vi "LabVIEW.Main.API_Test.vi"(7 "Chose Server":string, 8 "error in (no error)":errorcluster caption="Fehler (Eingang, kein Fehler)", 11 "result_folder_path":string) -> (0 "error out":errorcluster, 2 "Message_local_save":string, 3 "Message_report":string)   [LabVIEW 2026]
uses:
  LabVIEW.Type Definitions/LabVIEW.HTTPs_Client.Command.ctl
  LabVIEW.Type Definitions/LabVIEW.HTTPs_Client.Test_Group.Command.ctl
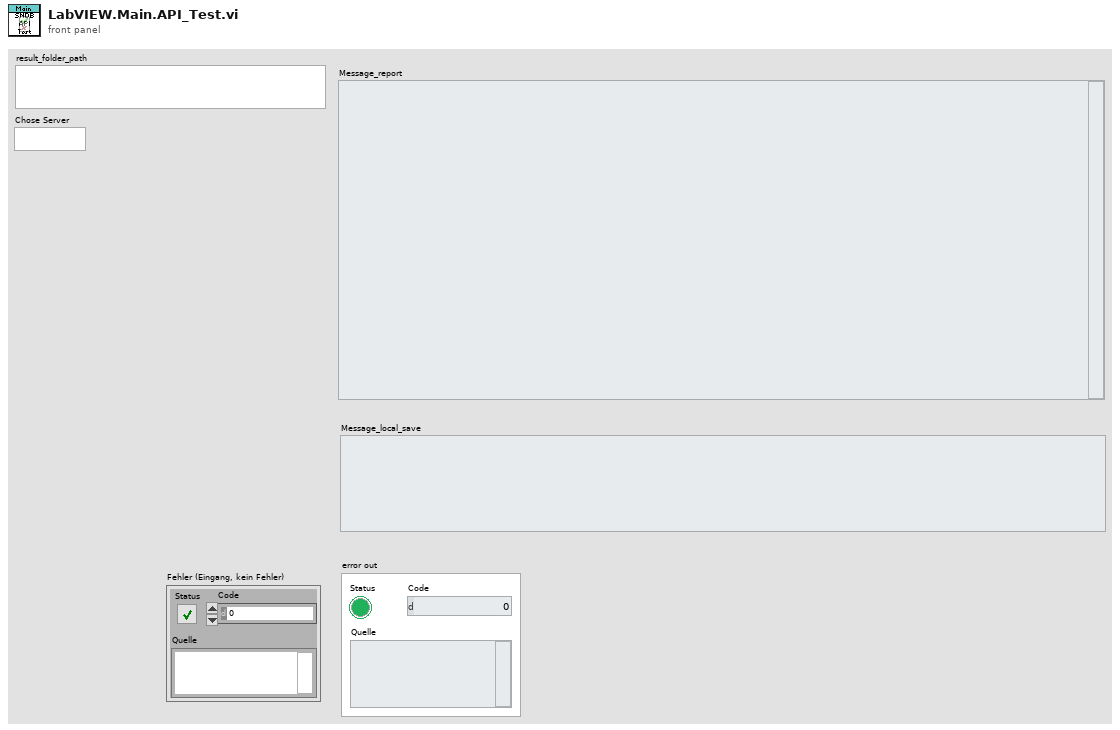
[diagram p1: front panel]
types:
  T1 = typedef "LabVIEW.HTTPs_Client.Command.ctl" = enum16{"Initialize HTTPS", "Authentication: Creat a token", "Authentication: Get all tokens", "Authentication: Revoke the token", "Label: Creat a label configuration", "Label: Get all configured labels", "Label: Update the label configuration", "Label: Delete the label configuration", "Label: Creat a colour ribbon", "Label: Update the colour ribbon", "Label: Get all colour ribbons", "Label: Delete the colour ribbon", "Label: Creat a label tape", "Label: Update the label tape", "Label: Get all label tapes", "Label: Delete the label tape", "Label: Get all label parameters", "Product: Get all product informations", "Product: Get all reading steps", "Seriennummer: Update the info text", "Seriennummer: Set all step states open", "Seriennummer: Update step states", "Seriennummer: Get data and steps", "Seriennummer: Get all label configurations", "Seriennummer: Create a text report(Prüfbericht)", "Seriennummer: Get the text report(Prüfbericht)", "Seriennummer: Delete the text report(Prüfbericht)", "Seriennummer: Upload a document(txt file)", "Seriennummer: Get the document", "Seriennummer: Get the document thumbnail", "Seriennummer: Delete the document", "Seriennummer: Bulk lookup", "Vorgang: Update the description text", "Vorgang: Migrate serial numbers to a Vorgang", "Vorgang: Migrate serial numbers to a product revision", "Vorgang: Update step states", "Vorgang: Create test reports(Prüfprotokoll)", "Vorgang: Get basic data", "Vorgang: Get serial number data and steps", "Vorgang: Get all serial numbers", "Vorgang: Generate a CSV file", "Vorgang: Generate an XLSX file", "Vorgang: Get a CSV file(Fertigmeldung report)", "Fertigmeldung: Create a Fertigmeldung", "Fertigmeldung: Revert the Fertigmeldung", "User: Get all users", "User: Update an user", "User: Get a single user", "User: Get all user roles", "User: Update a user role", "User: Get a single user role", "User: Get all permissions", "Search: Get Vorgang/Produkt combinations", "Search: Get Vorgang/Produkt/SN combinations", "Search: Get Seriennummern by Vorgang and Produkt", "Search: Lookup Vorgang", "MAC addresses: Get all reserved MAC addresses", "MAC addresses: Get the most recently reserved MAC addresses", "MAC addresses: Get data for a MAC address", "MAC addresses: Reserve MAC addresses for a Seriennummer", "MAC addresses: Mark a reserved MAC address as flashed", "Product: Get possible steps", "Product: Get all products", "Product: Create a new product", "Product: Update a product's data", "Product: Get next product IDs", "Product: Delete a product", "Product properties: Get all product property types", "Search: Find production plan", "Search: Find production plan arrangement", "Health check: Health check", "Deinitialize HTTPs"}
  T2 = typedef "LabVIEW.HTTPs_Client.Test_Group.Command.ctl" = enum16{"No Command", " Test Authentication in the beginning", "Test Label", "Test Seriennummer", "Test Vorgang/Fertigung/Search", "Test User/Role/Permission", "Test MAC addresses", "Test Product/Product properties", "Test Health check", " Test Authentication at the end"}
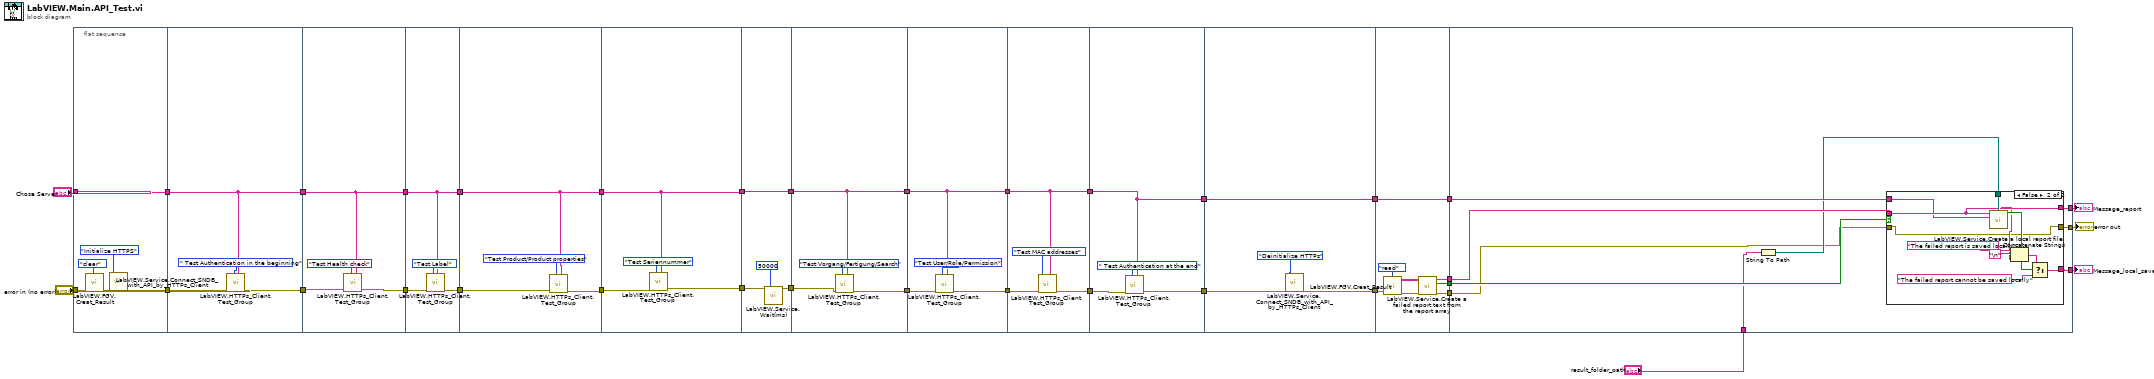
[diagram p0: block diagram]
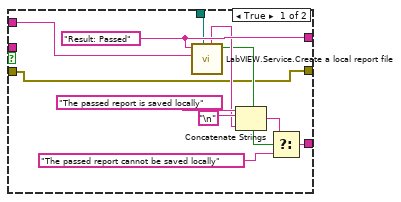
[diagram p2: hidden frame]
diagram:
  n1 = flat-sequence {
    tunnel: "error in (no error)" -> [w36]
    tunnel: [w39] -> w33
    tunnel: [w35] -> w19
    tunnel: "Chose Server" -> [w35]
    tunnel: w33 -> [w43]
    tunnel: [w42] -> w8
    tunnel: w19 -> [w41]
    tunnel: [w41] -> w6
    tunnel: w8 -> [w48]
    tunnel: [w47] -> w7
    tunnel: w6 -> [w45]
    tunnel: [w45] -> w5
    tunnel: w7 -> [w51]
    tunnel: [w50] -> w4
    tunnel: w5 -> [w49]
    tunnel: [w49] -> w2
    tunnel: w4 -> [w56]
    tunnel: [w55] -> w3
    tunnel: w2 -> [w53]
    tunnel: [w53] -> w1
    tunnel: w3 -> [w60]
    tunnel: [w59] -> w32
    tunnel: w1 -> [w58]
    tunnel: [w58] -> w17
    tunnel: w32 -> [w64]
    tunnel: [w63] -> w31
    tunnel: w17 -> [w61]
    tunnel: [w61] -> w16
    tunnel: w31 -> [w68]
    tunnel: [w67] -> w30
    tunnel: w16 -> [w65]
    tunnel: [w65] -> w15
    tunnel: w30 -> [w71]
    tunnel: [w70] -> w29
    tunnel: w15 -> [w69]
    tunnel: [w69] -> w14
    tunnel: w29 -> [w75]
    tunnel: [w74] -> w28
    tunnel: w14 -> [w73]
    tunnel: [w73] -> w13
    tunnel: w28 -> [w79]
    tunnel: [w78] -> w27
    tunnel: w13 -> [w77]
    tunnel: [w77] -> w10
    tunnel: w27 -> [w84]
    tunnel: [w82] -> w26
    tunnel: [w81] -> w11
    tunnel: w10 -> [w81]
    tunnel: w26 -> [w89]
    tunnel: [w88] -> w25
    tunnel: [w87] -> w24
    tunnel: [w86] -> w23
    tunnel: [w85] -> w12
    tunnel: w11 -> [w85]
    tunnel: w25 -> [w93]
    tunnel: w24 -> [w97]
    tunnel: w23 -> [w98]
    tunnel: [w101] -> w22
    tunnel: [w100] -> w21
    tunnel: [w99] -> w20
    tunnel: w12 -> [w96]
    tunnel: "result_folder_path" -> [w94]
    frame #0 {
      n2 = call "LabVIEW.FGV.Creat_Result.vi"("Command"=enum16{"write", "read", "clear"}."clear", "error in (no error)"=w36) -> ("error out"=w37:errorcluster)  [unwired: 8 in, 1 out]
      n3 = call "LabVIEW.Service.Connect_SNDB_with_API_by_HTTPs_Client.vi"("error in (no error)"=w37, "Command"=LabVIEW.HTTPs_Client.Command."Initialize HTTPS") -> ("error out"=w39:errorcluster)  [unwired: 15 in, 10 out]
    }
    frame #1 {
      n4 = call "LabVIEW.HTTPs_Client.Test_Group.vi"("Chose Server"=w41, "Command"=LabVIEW.HTTPs_Client.Test_Group.Command." Test Authentication in the beginning", "Fehler (Eingang, kein Fehler)"=w43) -> ("Fehler (Ausgang)"=w42:errorcluster)  [unwired: 8 in]
    }
    frame #2 {
      n5 = call "LabVIEW.HTTPs_Client.Test_Group.vi"("Chose Server"=w45, "Command"=LabVIEW.HTTPs_Client.Test_Group.Command."Test Health check", "Fehler (Eingang, kein Fehler)"=w48) -> ("Fehler (Ausgang)"=w47:errorcluster)  [unwired: 8 in]
    }
    frame #3 {
      n6 = call "LabVIEW.HTTPs_Client.Test_Group.vi"("Chose Server"=w49, "Command"=LabVIEW.HTTPs_Client.Test_Group.Command."Test Label", "Fehler (Eingang, kein Fehler)"=w51) -> ("Fehler (Ausgang)"=w50:errorcluster)  [unwired: 8 in]
    }
    frame #4 {
      n7 = call "LabVIEW.HTTPs_Client.Test_Group.vi"("Chose Server"=w53, "Command"=LabVIEW.HTTPs_Client.Test_Group.Command."Test Product/Product properties", "Fehler (Eingang, kein Fehler)"=w56) -> ("Fehler (Ausgang)"=w55:errorcluster)  [unwired: 8 in]
    }
    frame #5 {
      n8 = call "LabVIEW.HTTPs_Client.Test_Group.vi"("Chose Server"=w58, "Command"=LabVIEW.HTTPs_Client.Test_Group.Command."Test Seriennummer", "Fehler (Eingang, kein Fehler)"=w60) -> ("Fehler (Ausgang)"=w59:errorcluster)  [unwired: 8 in]
    }
    frame #6 {
      n9 = call "LabVIEW.Service.Wait(ms).vi"("milliseconds to wait (1000)"=u32 50000, "Error In (no error)"=w64) -> ("Error Out"=w63:errorcluster)  [unwired: 13 in]
    }
    frame #7 {
      n10 = call "LabVIEW.HTTPs_Client.Test_Group.vi"("Chose Server"=w65, "Command"=LabVIEW.HTTPs_Client.Test_Group.Command."Test Vorgang/Fertigung/Search", "Fehler (Eingang, kein Fehler)"=w68) -> ("Fehler (Ausgang)"=w67:errorcluster)  [unwired: 8 in]
    }
    frame #8 {
      n11 = call "LabVIEW.HTTPs_Client.Test_Group.vi"("Chose Server"=w69, "Command"=LabVIEW.HTTPs_Client.Test_Group.Command."Test User/Role/Permission", "Fehler (Eingang, kein Fehler)"=w71) -> ("Fehler (Ausgang)"=w70:errorcluster)  [unwired: 8 in]
    }
    frame #9 {
      n12 = call "LabVIEW.HTTPs_Client.Test_Group.vi"("Chose Server"=w73, "Command"=LabVIEW.HTTPs_Client.Test_Group.Command."Test MAC addresses", "Fehler (Eingang, kein Fehler)"=w75) -> ("Fehler (Ausgang)"=w74:errorcluster)  [unwired: 8 in]
    }
    frame #10 {
      n13 = call "LabVIEW.HTTPs_Client.Test_Group.vi"("Chose Server"=w77, "Command"=LabVIEW.HTTPs_Client.Test_Group.Command." Test Authentication at the end", "Fehler (Eingang, kein Fehler)"=w79) -> ("Fehler (Ausgang)"=w78:errorcluster)  [unwired: 8 in]
    }
    frame #11 {
      n14 = call "LabVIEW.Service.Connect_SNDB_with_API_by_HTTPs_Client.vi"("error in (no error)"=w84, "Command"=LabVIEW.HTTPs_Client.Command."Deinitialize HTTPs") -> ("error out"=w82:errorcluster)  [unwired: 15 in, 10 out]
    }
    frame #12 {
      n15 = call "LabVIEW.FGV.Creat_Result.vi"("Command"=enum16{"write", "read", "clear"}."read", "error in (no error)"=w89) -> ("error out"=w91:errorcluster, "Angehängtes Array"=w92:string[][])  [unwired: 8 in]
      n16 = call "LabVIEW.Service.Create a failed report text from the report array.vi"("error in (no error)"=w91, "Result[[]]"=w92) -> ("error out"=w88:errorcluster, "Passed?"=w87:bool, "report text"=w86:string)  [unwired: 7 in]
    }
    frame #13 {
      n17 = String To Path(string=w94) -> (path=w95:path)
      n18 = case shown="False" w97 {
        tunnel: w95 -> [w110 w123]
        tunnel: w98 -> [_ w119]
        tunnel: w93 -> [w102 w113]
        tunnel: [w103 w120] -> w101
        tunnel: [w112 w119] -> w100
        tunnel: [w102 w113] -> w99
        tunnel: w96 -> [w111 w114]
        frame True {
          w112 = "Result: Passed" ("report text")
          n19 = call "LabVIEW.Service.Create a local report file.vi"("Folder path"=w110, "Server type"=w111, "Failed report text"=w112) -> ("Successful?"=w104:bool, "Path"=w105:string)  [unwired: 6 in, 1 out]
          n20 = Concatenate Strings("The passed report is saved locally", "\n", w105) -> (w106:string)
          n21 = Select(t=w106, s=w104, f="The passed report cannot be saved locally") -> (s? t:f=w103:string)
        }
        frame False {
          n22 = call "LabVIEW.Service.Create a local report file.vi"("Folder path"=w123, "Server type"=w114, "Failed report text"=w119) -> ("Successful?"=w121:bool, "Path"=w116:string)  [unwired: 6 in, 1 out]
          n23 = Concatenate Strings("The failed report is saved locally", "\n", w116) -> (w115:string)
          n24 = Select(t=w115, s=w121, f="The failed report cannot be saved locally") -> (s? t:f=w120:string)
        }
      }
    }
  }
  "Message_report" <- w21
  "Message_local_save" <- w22
  "error out" <- w20
